vi "Dernier_element.vi"(0 "Tableau en entrée":dbl[](array[numeric])) -> (1 "Dernier élément":dbl, 2 "Indice N":i32, 3 "Taille/Indice N+1":i32)   [LabVIEW 2022 SP3]
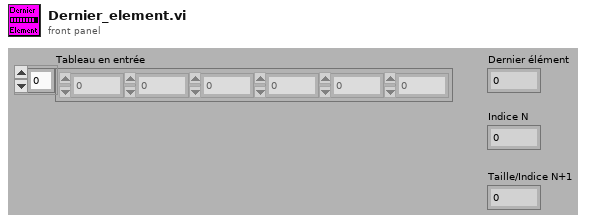
[diagram p1: front panel]
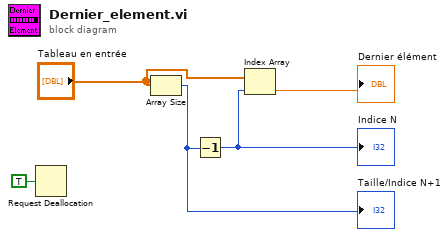
[diagram p0: block diagram]
diagram:
  n1 = Request Deallocation(TRUE ("flag")) -> ()
  n2 = Array Size(array="Tableau en entrée") -> (size(s)=w3:i32)
  "Taille/Indice N+1" <- w3
  n3 = Decrement(x=w3) -> (x-1=w2:i32)
  "Indice N" <- w2
  n4 = Index Array(array="Tableau en entrée", index=w2) -> (element=→"Dernier élément":dbl)
